vi "Load Parameters.vi"(8 "error in (no error)":errorcluster, 11 "Scheduler in":refnum<class "Scheduler.lvclass">) -> (0 "error out":errorcluster, 3 "Scheduler out":refnum<class "Scheduler.lvclass">)   [LabVIEW 2020, in "Scheduler.lvlib" / "Scheduler.lvclass"]
doc: "Load available parameters for each FPGA in the system"
uses:
  Scheduler.lvclass
  TALOS/TALOS_PPL.lvlibp/Support VIs/Global Memory.vi
  TALOS/TALOS_PPL.lvlibp/Interfaces/FPGA Interface/FPGA Interface.lvclass
  Scheduler.lvclass/Scheduler.ctl
  TALOS/TALOS_PPL.lvlibp
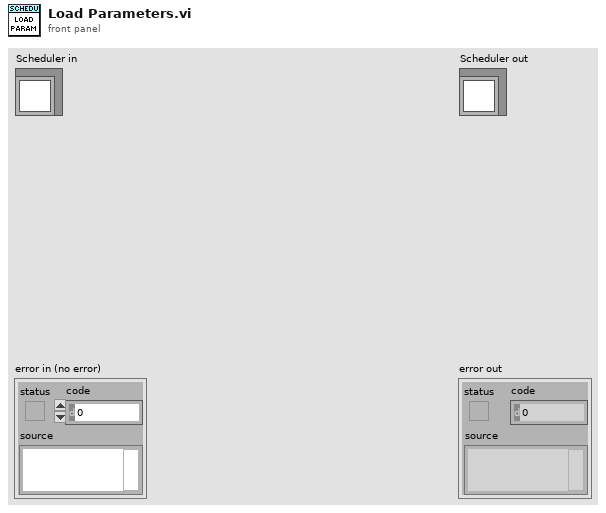
[diagram p1: front panel]
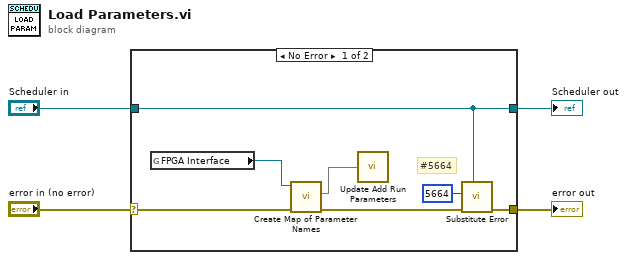
[diagram p0: block diagram]
diagram:
  n1 = case shown="No Error" "error in (no error)" {
    selector: "error in (no error)" -> [w9 w13]
    tunnel: [w11 w13] -> w3
    tunnel: [w6 w12] -> w1
    tunnel: "Scheduler in" -> [w6 w12]
    frame No Error {
      # "#5664"
      n2 = global read "Global Memory.vi" "FPGA Interface"() -> (w7:refnum<class "FPGA Interface.lvclass">)
      n3 = call-dynamic "Create Map of Parameter Names.vi"("error in (no error)"=w9, "FPGA Interface in"=w7) -> ("error out"=w8:errorcluster, "Parameters"=w5:map{string, string[]})  [unwired: 7 in, 1 out]
      n4 = call "Update Add Run Parameters.vi"("Parameters Map"=w5) -> ()
      n5 = call "Substitute Error.vi"("LabVIEW Object"=w6, "error in (no error)"=w8, "Error Code"=5664) -> ("error out"=w11:errorcluster)  [unwired: 8 in]
    }
    frame Error {
    }
  }
  "error out" <- w3
  "Scheduler out" <- w1
